vi "ReadAllOverlayGroups.vi"(8 "error in":errorcluster, 11 "Image Reference In":T1) -> (0 "error out":errorcluster, 2 "OverlayGroups":string[](array[string]), 3 "Image Reference Out":T1)   [LabVIEW 2020, in "OpenLvVision_Overlays.lvlib"]
doc: "Returns all overlay groups on an image."
uses:
  OpenLvVision_Overlays.lvlib
  <vilib>/OpenLvVision/OpenLvVision_Image/Management/TypeDef/OLV Image.ctl
  <vilib>/OpenLvVision/OpenLvVision_Image/Management/OLV Management.lvlib
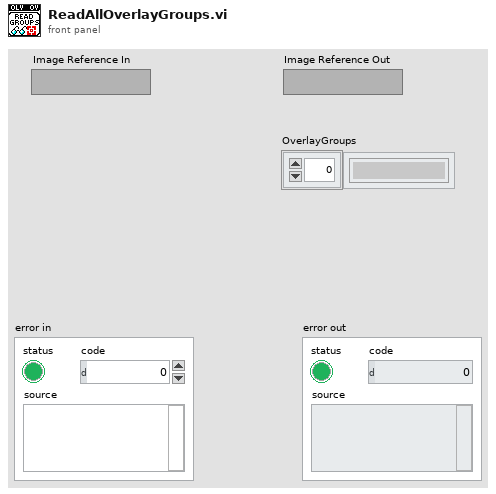
[diagram p1: front panel]
types:
  T1 = typedef "OLV OpenLvVision_Image.lvlib/OLV Management.lvlib/OLV Image.ctl" = refnum<image>
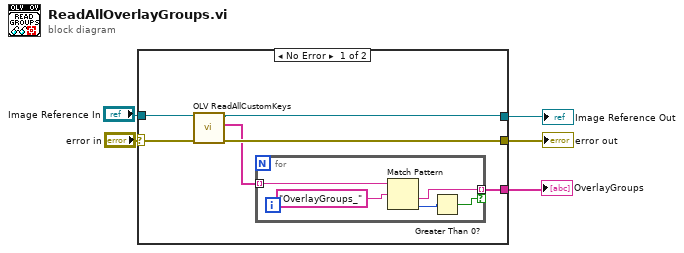
[diagram p0: block diagram]
diagram:
  n1 = case shown="No Error" "error in" {
    selector: "error in" -> [w11 w18]
    tunnel: [w8 w18] -> w4
    tunnel: [w9 w17] -> w3
    tunnel: "Image Reference In" -> [w10 w17]
    tunnel: [w6 _] -> w1
    frame No Error {
      n2 = call <vilib>:"OLV ReadAllCustomKeys.vi"("error in"=w11, "Image Reference In"=w10) -> ("error out"=w8:errorcluster, "Keys"=w7:string[], "Image Reference Out"=w9:T1)  [unwired: 6 in, 1 out]
      n3 = for {
        tunnel: w7 -> [w15] mode=indexing
        tunnel: [w13] -> w6 mode=indexing if=w14
        n4 = Match Pattern(string=w15, regular expression="OverlayGroups_" ("string")) -> (after substring=w13:string, offset past match=w16:i32)  [unwired: 1 in, 2 out]
        n5 = Greater Than 0?(x=w16) -> (x > 0?=w14:bool)
      }
    }
    frame Error {
    }
  }
  "error out" <- w4
  "Image Reference Out" <- w3
  "OverlayGroups" <- w1
